vi "PicoScope2000ExampleBlock.vi"() -> ()   [LabVIEW 2010]
uses:
  shared/PicoBuffers.ctl
  shared/Buffer and Transfer Settings.ctl
  shared/Acquisition Settings.ctl
  PicoScope2000Lib/PicoScope2000AnalogChannelSettings.ctl
panel:
  in  "Write to TDMS":bool
  in  "roundFaster":bool=TRUE
  in  "timeIntervalRequested":dbl min=0.0 format="%#6_6p"
  in  "Trigger Settings":T1={"Trigger Enabled"=FALSE, "Trigger Source"=enum."Channel A", "Trigger Threshold (V)"=0.0, "Trigger Direction"=0, "Trigger Delay (%)"=0, "Auto Trigger Time (ms)"=1000} {"Trigger Direction" items=["Rising", "Falling"]; "Trigger Threshold (V)" format="%.3f"}
  in  "Channel B Settings":T2={"Enabled"=TRUE, "Coupling"=1, "Range"=6} {"Range" items=["20 mV"=1, "50 mV"=2, "100 mV"=3, "200 mV"=4, "500 mV"=5, "1 V"=6, "2 V"=7, "5 V"=8, "10 V"=9, "20 V"=10]; "Coupling" items=["AC", "DC"]}
  in  "Channel A Settings":T2={"Enabled"=TRUE, "Coupling"=1, "Range"=7} {"Range" items=["20 mV"=1, "50 mV"=2, "100 mV"=3, "200 mV"=4, "500 mV"=5, "1 V"=6, "2 V"=7, "5 V"=8, "10 V"=9, "20 V"=10]; "Coupling" items=["AC", "DC"]}
  out "Unit Info":T3
  out "overflow":i16 format="%010b"
  in  "Apply Settings":bool
  out "error out":errorcluster
  in  "Data file":path=path "PicoScope2000ExampleBlock Data"
  in  "Buffer and Transfer Settings":T4={"startIndex"=0, "Samples"=3968, "Down Sample Ratio"=1, "Down-Sample Mode"=0} {"Down-Sample Mode" items=["RAW none"=2147483648, "None"=0, "Aggregate"=1, "Decimate"=2, "Average"=4]; "Down Sample Ratio" step=1; "Samples" format="%_6p"}
  in  "Acquisition Settings":T5={"preTriggerSamples"=0, "postTriggerSamples"=3968, "timebase"=0} {"postTriggerSamples" format="%_6p"; "preTriggerSamples" format="%_6p"}
  out "Properties Panel":T6 {"Max Total Capture Time Available (sec)" format="%.3p"; "Sample Frequency" format="%.6p"; "Sample Rate" format="%.3p"; "Max Samples Available" format="%_6p"; "Total Capture Time (sec)" format="%.3p"}
  in  "stop":bool
  out "Analog Channels":cluster{i32, dbl, "Data":dbl[]}[](graph)
  in  "error in (no error)":errorcluster
  # "Bit 0 = ChA"
  # "Oversample control ->"
  # "NOTE: Oversample ratio multiples the required device memory\nBuffer memory used = (pre+post trig samples) x Oversample"
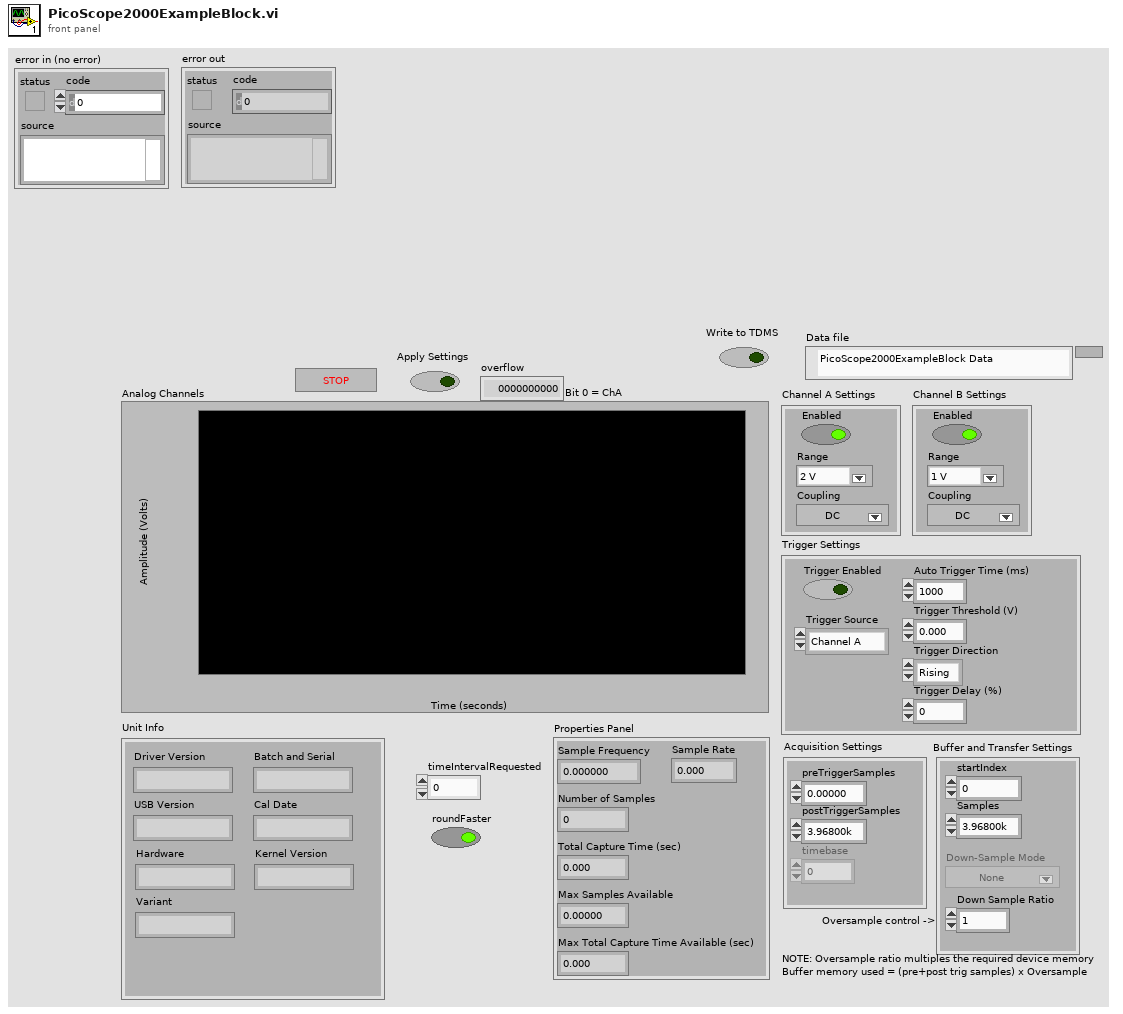
[diagram p1: front panel]
types:
  T1 = cluster{"Trigger Enabled":bool, "Trigger Source":enum16{"Channel A", "Channel B"}, "Trigger Threshold (V)":dbl, "Trigger Direction":i16, "Trigger Delay (%)":i16, "Auto Trigger Time (ms)":i16}
  T2 = typedef "PicoScope2000AnalogChannelSettings.ctl" = cluster{"Enabled":bool, "Coupling":i16, "Range":u16}
  T3 = cluster{"Driver Version":string, "USB Version":string, "Hardware":string, "Variant":string, "Batch and Serial":string, "Cal Date":string, "Kernel Version":string}
  T4 = typedef "Buffer and Transfer Settings.ctl" = cluster{"startIndex":u64, "Samples":u64, "Down Sample Ratio":u64, "Down-Sample Mode":u32}
  T5 = typedef "Acquisition Settings.ctl" = cluster{"preTriggerSamples":u64, "postTriggerSamples":u64, "timebase":u32}
  T6 = cluster{"Sample Frequency":dbl, "Sample Rate":dbl, "Max Samples Available":u64, "Number of Samples":u64, "Total Capture Time (sec) ":dbl, "Max Total Capture Time Available (sec)":dbl}
  T7 = typedef "PicoBuffers.ctl" = cluster{"Max Buffer Pointers":u64[][][], "Min Buffer Pointers":u64[][][], "StreamingDataInfo":cluster{"Channel":u32, "Down-Sample Mode":u32, "PICO_DATA_TYPE":enum32{"PICO_INT8_T", "PICO_INT16_T", "PICO_INT32_T", "PICO_UINT32_T", "PICO_INT64_T", ""}, "Samples":i32, "bufferIndex":u64, "startIndex":i32, "overflow":i16}[][]}
  T8 = enum16{"open", "open or create", "create or replace", "create", "open (read-only)"}
  T9 = cluster{"Sample Frequency":sgl, "Sample Rate":sgl, "Max Samples Available":i32, "Number of Samples":u32, "Total Capture Time (sec) ":sgl, "Max Total Capture Time Available (sec)":sgl}
  T10 = cluster{"Channel A Buffer":i16[], "Channel B Buffer":i16[], "Channel C Buffer":i16[], "Channel D Buffer":i16[], "Channel E Buffer":i16[], "Channel F Buffer":i16[], "Channel G Buffer":i16[], "Channel H Buffer":i16[], "Port 0 Buffer":i16[], "Port 1 Buffer":i16[]}[]
  T11 = cluster{"Channel A Buffer":i16[], "Channel B Buffer":i16[], "Channel C Buffer":i16[], "Channel D Buffer":i16[], "Channel E Buffer":i16[], "Channel F Buffer":i16[], "Channel G Buffer":i16[], "Channel H Buffer":i16[], "Port 0 Buffer":i16[], "Port 1 Buffer":i16[]}
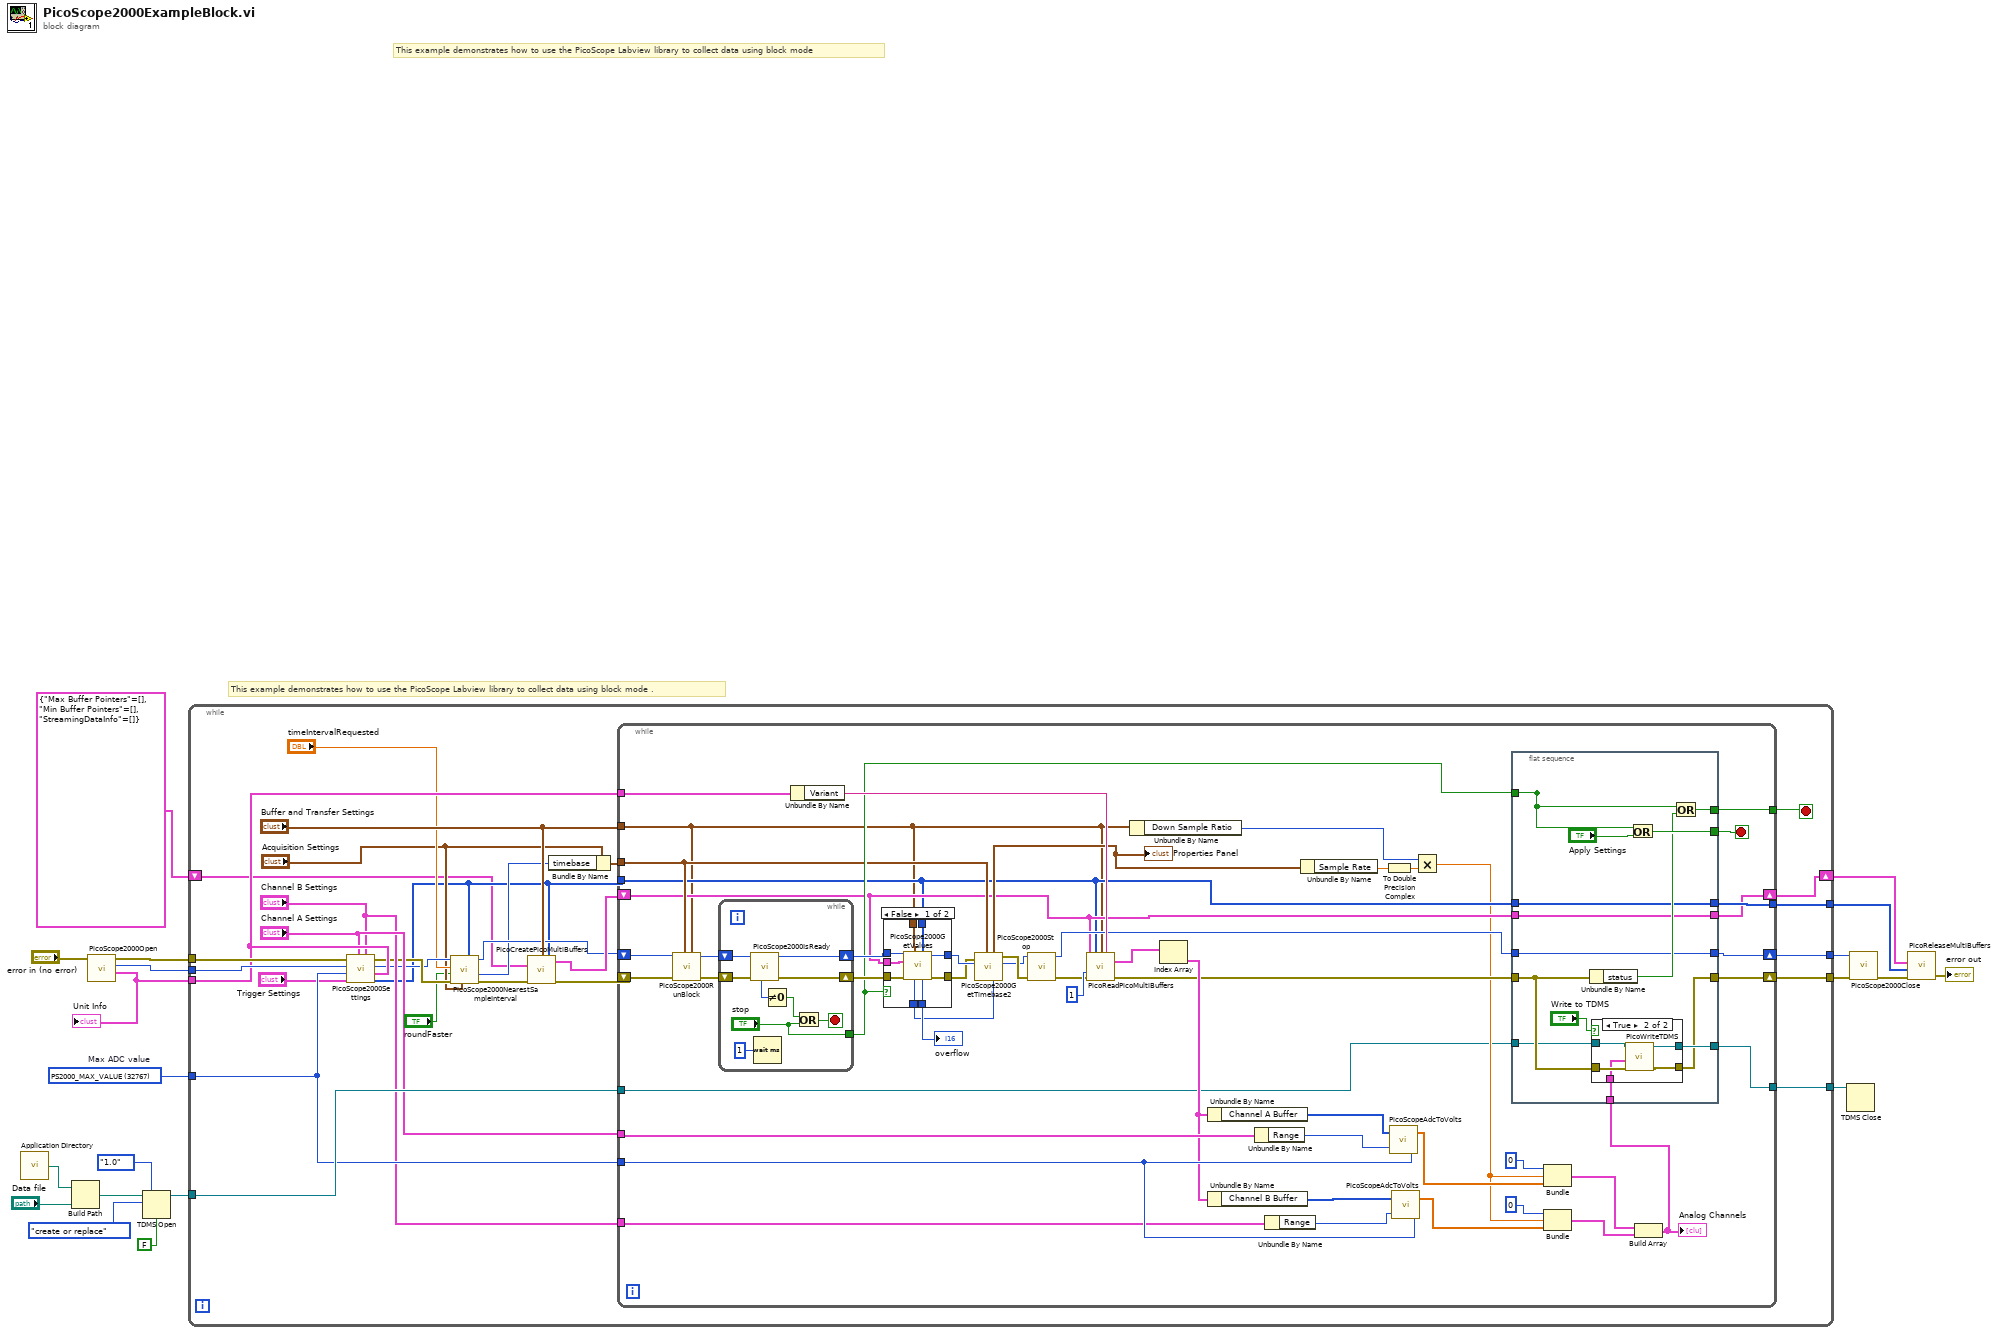
[diagram p0: block diagram]
diagram:
  w3 = i16 32767 items=["PS2000_MAX_VALUE"=32767]  # Max ADC value
  # "This example demonstrates how to use the PicoScope Labview library to collect data using block mode ."
  # "This example demonstrates how to use the PicoScope Labview library to collect data using block mode"
  n1 = call <vilib>:"Application Directory.vi"() -> ("Application Directory"=w14:path)
  n2 = Build Path(base path=w14, name or relative path="Data file") -> (appended path=w15:path)
  n3 = call "PicoScope2000Open.vi"("error in (no error)"="error in (no error)") -> ("Unit Info"=w6:T3, "handle"=w7:i16, "error out"=w8:errorcluster)  [unwired: 6 in]
  "Unit Info" <- w6
  n4 = TDMS Open(6:FALSE ("disable buffering? (T)"), 7:enum16{"1.0", "2.0"}."1.0" ("file format version (2.0)"), 10:T8."create or replace" ("operation (0:open)"), 11:w15) -> (3:w12:refnum<k34>)  [unwired: 2 in, 1 out]
  n5 = while {
    tunnel: w7 -> [w46]
    tunnel: w3 -> [w40]
    tunnel: [w33] -> w20
    tunnel: [w43] -> w13
    tunnel: w12 -> [w47]
    tunnel: w6 -> [w39]
    tunnel: w8 -> [w45]
    tunnel: [w44] -> w4
    tunnel: [w41] -> w5
    shift-right: [w21] -> w1
    shift-left: T7 {"Max Buffer Pointers"=[], "Min Buffer Pointers"=[], "StreamingDataInfo"=[]} ("Data Pointers") -> [w22]
    stop <- w42 stop-if-true
    n6 = call "PicoScope2000Settings.vi"("Unit Info"=w39, "Channel B Settings"="Channel B Settings", "Channel A Settings"="Channel A Settings", "Trigger Settings"="Trigger Settings", "Max ADC value"=w40, "handle in"=w46, "error in"=w45) -> ("Enabled Array"=w23:i16[], "handle out"=w29:i16, "error out"=w32:errorcluster)
    n7 = call "PicoScope2000NearestSampleInterval.vi"("Enabled Array"=w23, "Acquisition Settings"="Acquisition Settings", "error in (no error)"=w32, "roundFaster"="roundFaster", "timeIntervalRequested"="timeIntervalRequested", "handle in"=w29) -> ("error out"=w31:errorcluster, "timebase"=w27:i16, "handle out"=w30:i16)  [unwired: 2 in, 1 out]
    n8 = call "PicoCreatePicoMultiBuffers.vi"("Buffer and Transfer Settings"="Buffer and Transfer Settings", "enabled array"=w23, "Data Pointers In"=w22, "error in (no error)"=w31) -> ("Data Pointers"=w48:T7, "error out"=w37:errorcluster)  [unwired: 10 in]
    n9 = Bundle By Name(cluster="Acquisition Settings", "timebase"=w27) -> (w26:T5)
    n10 = while {
      tunnel: "Buffer and Transfer Settings" -> [w56]
      tunnel: w23 -> [w65]
      tunnel: "Channel A Settings" -> [w97]
      tunnel: w26 -> [w71]
      tunnel: w40 -> [w96]
      tunnel: w39 -> [w94]
      tunnel: [w80] -> w42
      shift-right: [w82] -> w44
      shift-left: w37 -> [w63]
      shift-right: [w78] -> w41
      shift-left: w30 -> [w62]
      tunnel: w47 -> [w51]
      tunnel: [w53] -> w43
      tunnel: "Channel B Settings" -> [w72]
      tunnel: [w66] -> w33
      shift-right: [w54] -> w21
      shift-left: w48 -> [w67]
      stop <- w79 stop-if-true
      n11 = call "PicoScope2000RunBlock.vi"("Buffer and Transfer Settings"=w56, "Acquisition Settings"=w71, "error in (no error)"=w63, "handle in"=w62) -> ("error out"=w99:errorcluster, "handle out"=w98:i16)  [unwired: 4 in, 2 out]
      n12 = while {
        shift-right: [w140] -> w76
        shift-left: w99 -> [w141]
        shift-right: [w139] -> w77
        shift-left: w98 -> [w138]
        tunnel: ["stop"] -> w75
        stop <- w135 stop-if-true
        n13 = call "PicoScope2000IsReady.vi"("error in (no error)"=w141, "handle in"=w138) -> ("error out"=w140:errorcluster, "handle out"=w139:i16, "ready"=w137:i16)  [unwired: 7 in]
        n14 = Wait (ms)(milliseconds to wait=u32 1) -> ()  [unwired: 1 out]
        n15 = Not Equal To 0?(x=w137) -> (x != 0?=w136:bool)
        n16 = Or(x=w136, y="stop") -> (x .or. y?=w135:bool)
      }
      n17 = Unbundle By Name(w94) -> ("Variant"=w95:string)
      n18 = case shown="False" w75 {
        tunnel: w76 -> [w109 w110]
        tunnel: w77 -> [w108 w111]
        tunnel: [w107 w111] -> w61
        tunnel: [w106 w110] -> w60
        tunnel: [w105 _] -> w74
        tunnel: [w104 _] -> w64
        tunnel: w65 -> [w103 _]
        tunnel: w67 -> [w102 _]
        tunnel: w56 -> [w101 _]
        frame False {
          n19 = call "PicoScope2000GetValues.vi"("enabled array"=w103, "Buffer and Transfer Settings"=w101, "error in (no error)"=w109, "Data Pointers In"=w102, "handle in"=w108) -> ("error out"=w106:errorcluster, "handle out"=w107:i16, "overflow"=w105:i16, "noOfSamples"=w104:u64)  [unwired: 3 in]
        }
        frame True {
        }
      }
      "overflow" <- w74
      n20 = call "PicoScope2000GetTimebase2.vi"("Number of Samples"=w64, "Acquisition Settings"=w71, "handle in"=w61, "error in (no error)"=w60) -> ("handle out"=w58:i16, "error out"=w59:errorcluster, "Properties Panel"=w70:T9)  [unwired: 5 in]
      "Properties Panel" <- w70
      n21 = call "PicoScope2000Stop.vi"("error in (no error)"=w59, "handle in"=w58) -> ("error out"=w69:errorcluster, "handle out"=w68:i16)  [unwired: 8 in]
      n22 = call "PicoReadPicoMultiBuffers.vi"("enabled array"=w65, "Buffer and Transfer Settings"=w56, "Variant"=w95, "Data Pointers"=w67, "No of Buffers"=1, "error in (no error)"=w69) -> ("MultiBuffers (Max or non-aggregated)"=w100:T10, "error out"=w81:errorcluster)  [unwired: 7 in, 1 out]
      n23 = Unbundle By Name(w56) -> ("Down Sample Ratio"=w55:u64)
      n24 = Index Array(array=w100) -> (element=w83:T11)  [unwired: 1 in]
      n25 = Unbundle By Name(w83) -> ("Channel A Buffer"=w84:i16[])
      n26 = Unbundle By Name(w83) -> ("Channel B Buffer"=w89:i16[])
      n27 = Unbundle By Name(w97) -> ("Range"=w91:u16)
      n28 = Unbundle By Name(w72) -> ("Range"=w73:u16)
      n29 = Unbundle By Name(w70) -> ("Sample Rate"=w49:sgl)
      n30 = To Double Precision Complex(1:w49) -> (0:w50:cdb)
      n31 = call "PicoScopeAdcToVolts.vi"("Max_adc"=w96, "Range Index"=w91, "Data"=w84) -> ("Data"=w85:dbl[])
      n32 = call "PicoScopeAdcToVolts.vi"("Max_adc"=w96, "Range Index"=w73, "Data"=w89) -> ("Data"=w88:dbl[])
      n33 = Multiply(x=w55, y=w50) -> (x*y=w57:cdb)
      n34 = flat-sequence {
        tunnel: [w125] -> w79
        tunnel: [w120] -> _
        tunnel: [w122] -> w80
        tunnel: w68 -> [w121]
        tunnel: [w121] -> w78
        tunnel: w81 -> [w114]
        tunnel: [w115] -> w82
        tunnel: w75 -> [w120]
        tunnel: w67 -> [w119]
        tunnel: [w119] -> w54
        tunnel: [w118] -> w66
        tunnel: w65 -> [w118]
        tunnel: [w116] -> w53
        tunnel: w52 -> [w113]
        tunnel: w51 -> [w112]
        frame #0 {
          n35 = Unbundle By Name(w114) -> ("status"=w123:bool)
          n36 = case shown="True" "Write to TDMS" {
            tunnel: [w127 w132] -> w116
            tunnel: [w126 w131] -> w115
            tunnel: w114 -> [w126 w130]
            tunnel: w113 -> [_ w129]
            tunnel: w112 -> [w127 w128]
            frame False {
            }
            frame True {
              n37 = call "PicoWriteTDMS.vi"("error in (no error)"=w130, "Analog Channels"=w129, "Refnum in"=w128) -> ("error out"=w131:errorcluster, "Refnum out"=w132:refnum<k34>)  [unwired: 7 in]
            }
          }
          n38 = Or(x=w120, y="Apply Settings") -> (x .or. y?=w125:bool)
          n39 = Or(x=w120, y=w123) -> (x .or. y?=w122:bool)
        }
      }
      n40 = Bundle(0, w57, "Data"=w85) -> (w87:cluster{i32, cdb, "Data":dbl[]})  [unwired: 1 in]
      n41 = Bundle(0, w57, "Data"=w88) -> (w86:cluster{i32, cdb, "Data":dbl[]})  [unwired: 1 in]
      n42 = Build Array(w87, w86) -> (w52:cluster{i32, cdb, "Data":dbl[]}[])
      "Analog Channels" <- w52
    }
  }
  n43 = TDMS Close(11:w13) -> ()  [unwired: 1 in, 2 out]
  n44 = call "PicoScope2000Close.vi"("error in"=w4, "handle"=w5) -> ("error out"=w9:errorcluster)  [unwired: 4 in, 1 out]
  n45 = call "PicoReleaseMultiBuffers.vi"("error in (no error)"=w9, "Enabled array"=w20, "Data Pointers"=w1) -> ("error out"=→"error out":errorcluster)  [unwired: 7 in, 1 out]
